vi "test--Cyan.vi"(11 "Test Case In":refnum<class "HSL to Color.lvclass">) -> (0 "error out":errorcluster, 3 "Test Case Out":refnum<class "HSL to Color.lvclass">)   [LabVIEW 2021, in "HSL to Color.lvclass"]
uses:
  HSL to Color.lvclass
  C:/Program Files/National Instruments/LabVIEW 2026/vi.lib/Astemes/LUnit/Test Case.lvclass
  <vilib>/Astemes/LUnit/Test Case.lvclass/Test Case.ctl
  21945745-6a43-4f25-9869-c7df3bc0736d.vi
  src/Material SubVIs/tsc--RGB to Color.vi
  <vilib>/Astemes/LUnit/Core/LUnit Test Case/Private/Append Pass Result.vi
  <vilib>/Astemes/LUnit/Core/LUnit Test Case/Private/Append Fail Result.vi
  21945745-6a43-4f25-9869-c7df3bc0736d.vi/9c5d11cd-9439-4240-a1ee-d9baace9c924.vi
  <vilib>/Astemes/LUnit/Core/LUnit Test Case/Private/Run In UI.vi
  <vilib>/Utility/error.llb/Clear Errors.vi
  src/Material SubVIs/Material SubVIs.lvlib
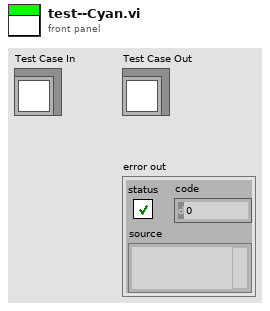
[diagram p1: front panel]
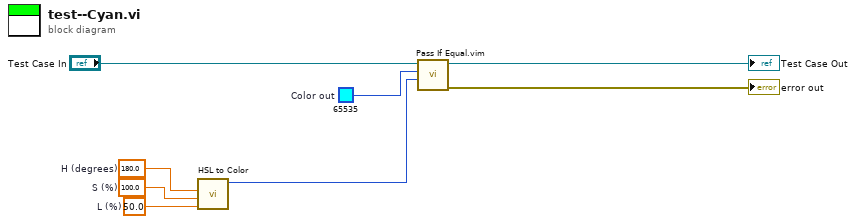
[diagram p0: block diagram]
diagram:
  w3 = 180.0  # H (degrees)
  w4 = 100.0  # S (%)
  w5 = 50.0  # L (%)
  w2 = u32 65535  # Color out
  n1 = call "HSL to Color.vi"("L (%)"=w5, "S (%)"=w4, "H (degrees)"=w3) -> ("Color out"=w1:u32)  [unwired: 5 in, 3 out]
  n2 = call "Pass If Equal.vim"("Actual"=w1, "Expected"=w2, "LUnit Test Case In"="Test Case In") -> ("error out"=→"error out":errorcluster, "LUnit Test Case Out"=→"Test Case Out":refnum<class "HSL to Color.lvclass">)  [unwired: 7 in]
